vi "Day 17.vi"() -> ()   [LabVIEW 2021]
uses:
  7ab77bb0-e42a-4831-84bc-49c84d93f386.vi
  <vilib>/Utility/file.llb/Read Delimited Spreadsheet (I64).vi
  <vilib>/Comparison/Less/Less Functor/Less Functor.lvclass
panel:
  out "Possible Initial Velocities":cluster{i64, i64}[](array[cluster])
  out "Input":i64[](array[numeric])
  in  "Input File":enum32{"example input", "input"}(radio)
  out "Possibilities":i16
  out "Max y":i64
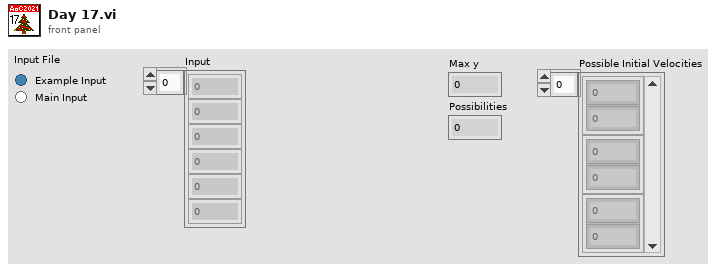
[diagram p1: front panel]
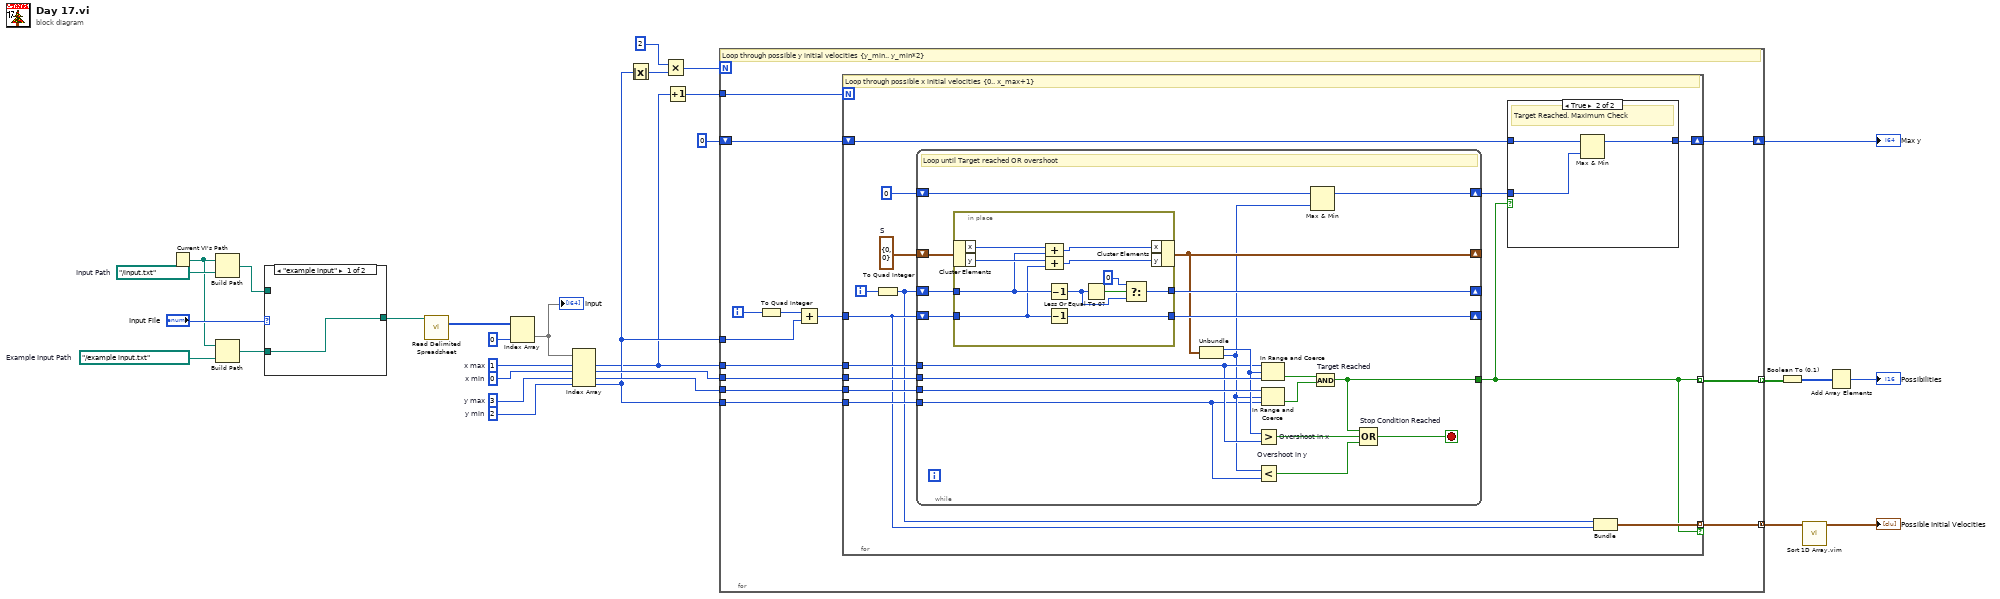
[diagram p0: block diagram]
diagram:
  w10 = 2  # y min
  w11 = 3  # y max
  w13 = 0  # x min
  w14 = 1  # x max
  w23 = path "../example input.txt"  # Example Input Path
  w24 = path "../input.txt"  # Input Path
  n1 = Current VI's Path() -> (path=w18:path)
  n2 = Build Path(base path=w18, name or relative path=w24) -> (appended path=w21:path)
  n3 = Build Path(base path=w18, name or relative path=w23) -> (appended path=w20:path)
  n4 = case shown="\"example input\"" "Input File" {
    tunnel: w21 -> [_ w31]
    tunnel: w20 -> [w30 _]
    tunnel: [w30 w31] -> w19
    frame "example input" {
    }
    frame "input" {
    }
  }
  n5 = call-poly <vilib>:"Read Delimited Spreadsheet.vi"("file path (dialog if empty)"=w19) -> ("all rows"=w17:i64[][])  [unwired: 9 in, 5 out]
  n6 = Index Array(array=w17, index (col)=0 ("disabled index (col)")) -> (element=w15:i64[])  [unwired: 1 in]
  "Input" <- w15
  n7 = Index Array(array=w15, index #1=w14, index #2=w13, index #3=w11, index #4=w10) -> (element #1=w7:i64, element #2=w12:i64, element #3=w9:i64, element #4=w8:i64)
  n8 = Absolute Value(x=w8) -> (abs(x)=w5:i64)
  n9 = Multiply(x=i64 2, y=w5) -> (x*y=w4:i64)
  n10 = Increment(x=w7) -> (x+1=w6:i64)
  n11 = for {
    N: w4 -> [_]
    tunnel: w7 -> [w44]
    tunnel: w12 -> [w43]
    tunnel: w9 -> [w42]
    tunnel: w8 -> [w41]
    shift-right: [w39] -> w28
    shift-left: i64 0 -> [w40]
    tunnel: [w33] -> w27 mode=indexing
    tunnel: w8 -> [w37]
    tunnel: w6 -> [w36]
    tunnel: [w34] -> w2 mode=concatenating
    i -> [w38]
    # "Loop through possible y initial velocities {y_min.. y_min*2}"
    n12 = To Quad Integer(1:w38) -> (0:w35:i64)
    n13 = Add(x=w35, y=w37) -> (x+y=w32:i64)
    n14 = for {
      N: w36 -> [_]
      tunnel: w32 -> [w48]
      tunnel: w44 -> [w57]
      tunnel: w43 -> [w56]
      tunnel: w42 -> [w55]
      tunnel: w41 -> [w54]
      shift-right: [w50] -> w39
      shift-left: w40 -> [w52]
      tunnel: [w46] -> w33 mode=indexing
      tunnel: [w47] -> w34 mode=indexing if=w46
      i -> [w49]
      w58 = cluster{"x":i64, "y":i64} {"x"=0, "y"=0}  # S
      # "Loop through possible x initial velocities {0.. x_max+1}"
      n15 = To Quad Integer(1:w49) -> (0:w45:i64)
      n16 = while {
        shift-right: [w72] -> _
        shift-left: w58 -> [w74]
        shift-right: [w76] -> _
        shift-left: w45 -> [w78]
        shift-right: [w75] -> _
        shift-left: w48 -> [w77]
        tunnel: w57 -> [w66]
        tunnel: w56 -> [w71]
        tunnel: w55 -> [w69]
        tunnel: w54 -> [w60]
        shift-right: [w63] -> w51
        shift-left: 0 -> [w62]
        tunnel: [w59] -> w46
        stop <- w73 stop-if-true
        # "Loop until Target reached OR overshoot"
        n17 = in-place {
          in-place-border: w78 -> [w85]
          in-place-border: w77 -> [w80]
          in-place-border: [w81] -> w76
          in-place-border: [w79] -> w75
          n18 = in-place-cluster #1(w74) -> ("x"=w89:i64, "y"=w88:i64)
          n19 = Compound Arithmetic op=ADD(w89, w85) -> (w87:i64)
          n20 = Compound Arithmetic op=ADD(w88, w80) -> (w86:i64)
          n21 = Decrement(x=w85) -> (x-1=w82:i64)
          n22 = Decrement(x=w80) -> (x-1=w79:i64)
          n23 = Less Or Equal To 0?(x=w82) -> (x <= 0?=w84:bool)
          n24 = Select(t=i64 0, s=w84, f=w82) -> (s? t:f=w81:i64)
          n25 = in-place-cluster #1("x"=w87, "y"=w86) -> (w72:cluster{"x":i64, "y":i64})
        }
        n26 = Unbundle(w72) -> ("x"=w67:i64, "y"=w61:i64)
        n27 = Greater? "Overshoot in x"(x=w67, y=w66) -> (0:w65:bool)
        n28 = Less? "Overshoot in y"(x=w61, y=w60) -> (x < y?=w64:bool)
        n29 = In Range and Coerce(upper limit=w66, x=w67, lower limit=w71) -> (In Range?=w70:bool)  [unwired: 1 out]
        n30 = In Range and Coerce(upper limit=w69, x=w61, lower limit=w60) -> (In Range?=w68:bool)  [unwired: 1 out]
        n31 = Max & Min(x=w62, y=w61) -> (max(x,y)=w63:i64)  [unwired: 1 out]
        n32 = Compound Arithmetic op=AND "Target Reached"(w70, w68) -> (w59:bool)
        n33 = Compound Arithmetic op=OR "Stop Condition Reached"(w59, w65, w64) -> (w73:bool)
      }
      n34 = case shown="True" w46 {
        tunnel: w52 -> [w90 w93]
        tunnel: w51 -> [_ w92]
        tunnel: [w90 w91] -> w50
        frame False {
          # "Target not Reached"
        }
        frame True {
          # "Target Reached. Maximum Check"
          n35 = Max & Min(x=w93, y=w92) -> (max(x,y)=w91:i64)  [unwired: 1 out]
        }
      }
      n36 = Bundle(w45, w48) -> (w47:cluster{i64, i64})  [unwired: 1 in]
    }
  }
  "Max y" <- w28
  n37 = Boolean To (0,1)(Boolean=w27) -> (0, 1=w26:i16[][])
  n38 = call "Sort 1D Array.vim"("unsorted array"=w2) -> ("sorted array"=→"Possible Initial Velocities":cluster{i64, i64}[])  [unwired: 10 in]
  n39 = Add Array Elements(numeric array=w26) -> (sum=→"Possibilities":i16)
